vi "PicoScope4000UnitInfo.vi"(7 "Mode":u16(ring) items=["Dialog On Error", "no dialog - CloseUnit and Stop", "no dialog - Continue", "no dialog - Stop"], 8 "error in (no error)":errorcluster, 11 "handle in":i16) -> (0 "error out":errorcluster, 1 "Unit Info":T1, 2 "requiredSize":i16[](array[numeric]), 3 "handle out":i16)   [LabVIEW 2010]
uses:
  ps4000.dll
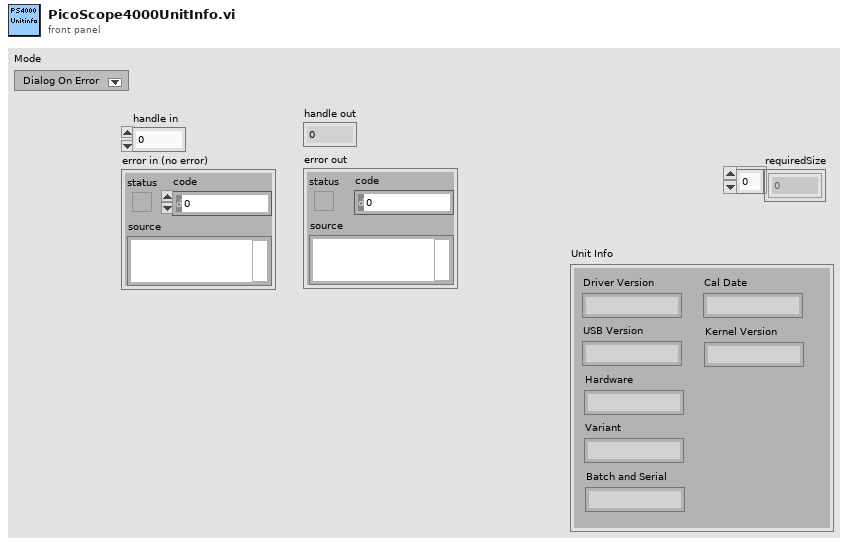
[diagram p1: front panel]
types:
  T1 = cluster{"Driver Version":string, "USB Version":string, "Hardware":string, "Variant":string, "Batch and Serial":string, "Cal Date":string, "Kernel Version":string}
  T2 = cluster{"status":bool, "code":u32, "source":string}
  T3 = cluster{"[0]":string, "[1]":string, "[2]":string, "[3]":string, "[4]":string, "[5]":string, "[6]":string}
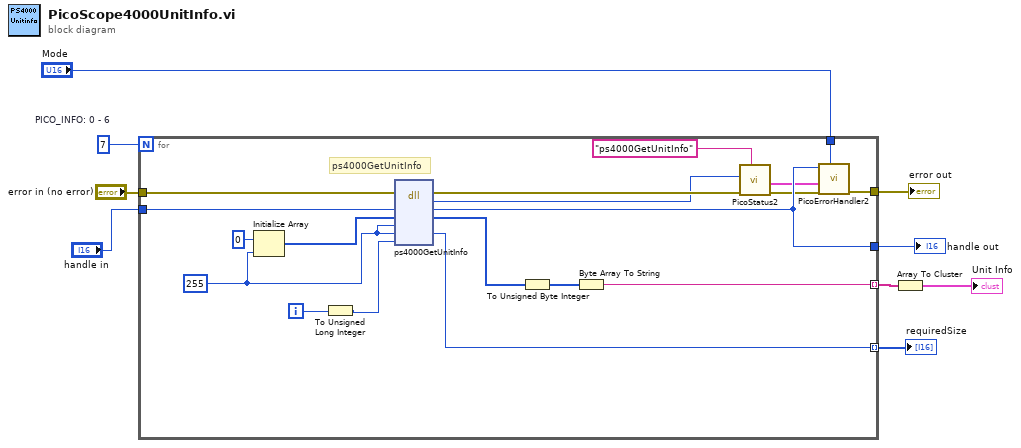
[diagram p0: block diagram]
diagram:
  w8 = 7  # PICO_INFO: 0 - 6
  n1 = for {
    N: w8 -> [_]
    tunnel: "handle in" -> [w28]
    tunnel: [w19] -> w6 mode=indexing
    tunnel: "error in (no error)" -> [w27]
    tunnel: [w26] -> w3
    tunnel: [w20] -> w4 mode=indexing
    tunnel: [w16] -> w2
    tunnel: "Mode" -> [w10]
    i -> [w22]
    w23 = i16 255 ("requiredSize")
    # "ps4000GetUnitInfo"
    n2 = Initialize Array(i8 0 ("element"), w23) -> (w24:i8[])
    n3 = To Unsigned Long Integer(number=w22) -> (unsigned 32bit integer=w21:u32)
    n4 = dll-call lib="ps4000.dll" fn="ps4000GetUnitInfo"(error in=w27, "handle"=w28, "stringUnitInfo"=w24, "stringLength"=w23, "requiredSize"=w23, "pico_info"=w21) -> (error out=w12:errorcluster, "PICO_STATUS"=w11:u32, "handle"=w26:i16, "stringUnitInfo"=w17:i8[], "requiredSize"=w20:i16)  [unwired: 4 in, 1 out]
    n5 = To Unsigned Byte Integer(number=w17) -> (unsigned 8bit integer=w18:u8[])
    n6 = Byte Array To String(unsigned byte array=w18) -> (string=w19:string)
    n7 = call "PicoStatus2.vi"("PICO source"="ps4000GetUnitInfo" ("source"), "Error in"=w12, "PICO STATUS"=w11) -> ("error out"=w15:errorcluster, "PICO_STATUS out"=w14:T2)  [unwired: 5 in]
    n8 = call "PicoErrorHandler2.vi"("Mode"=w10, "error in (no error)"=w15, "PICO_STATUS in"=w14, "handle In"=w26) -> ("error out"=w16:errorcluster)  [unwired: 7 in]
  }
  "error out" <- w2
  "handle out" <- w3
  "requiredSize" <- w4
  n9 = Array To Cluster(array=w6) -> (cluster=→"Unit Info":T3)
